vi "Func - Get list of string arguments.vi"(5 "InstanceRef":T1, 6 "error in":bool, 7 "max arg num":i32=100, 8 "min arg num":i32=1, 9 "arg list":T2[](array[typedef])) -> (0 "error out":bool, 3 "val list":string[](array[string]))   [LabVIEW 2021]
doc: "This VI returns the values of function arguments which must all have the <b>String</b> data type. It verifies the number of actual arguments and their data types. Refer to the VI help for more details.\n\n<b>arg list</b> specifies the list of function arguments passed to a FuncVI. Wire it to the same terminal on the FuncVI block diagram.\n\n<b>min arg num</b> and <b>max arg num</b> specify the minimum and the maximum number of arguments allowed.\n\n::: CalcExpress Toolkit :::\nCopyright (c) 2000-2026 Konstantin Shifershteyn. All rights reserved."
uses:
  cetypes.llb/CalcExpress Function Argument Info.ctl
  cetypes.llb/CalcExpress Instance RefNum.ctl
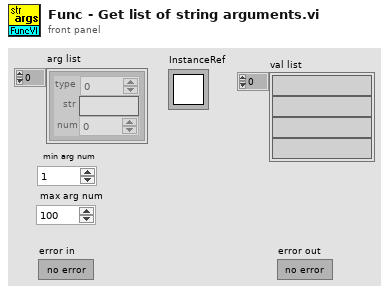
[diagram p1: front panel]
types:
  T1 = typedef "CalcExpress Instance RefNum.ctl" = refnum<k1>
  T2 = typedef "CalcExpress Function Argument Info.ctl" = cluster{"type":u32, "str":string, "num":dbl}
  T3 = enum32{"String", "DBL Number", "identifier", "1D Array of DBL", "2D Array of DBL", "CDB Number", "1D Array of CDB", "2D Array of CDB", "1D Array of String", "2D Array of String", "Unknown data type"}
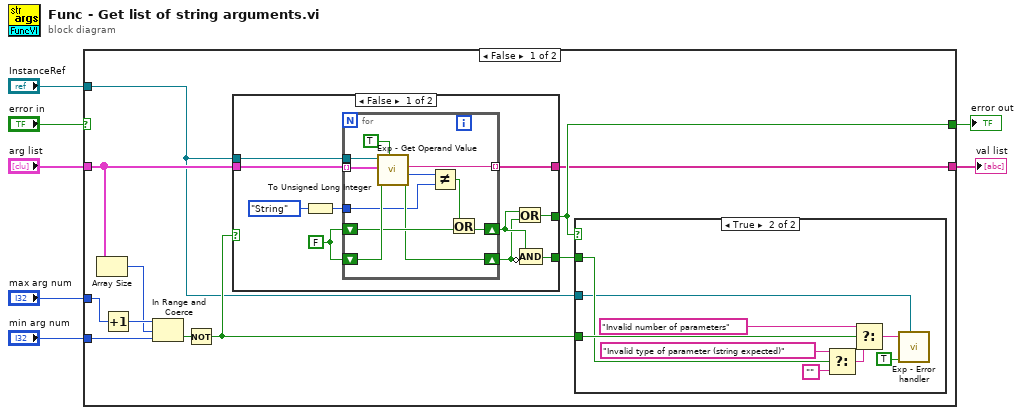
[diagram p0: block diagram]
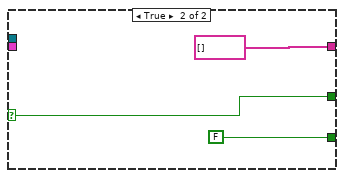
[diagram p2: hidden frame]
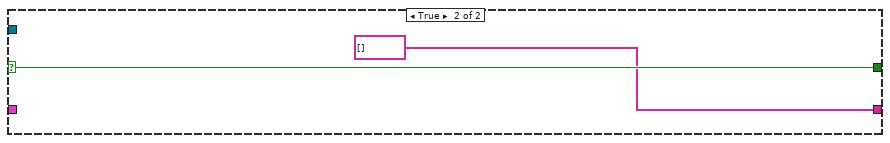
[diagram p4: hidden frame]
diagram:
  n1 = case shown="False" "error in" {
    selector: "error in" -> [_ w53]
    tunnel: [w13 w53] -> w7
    tunnel: [w12 string[] []] -> w6
    tunnel: "InstanceRef" -> [w8 _]
    tunnel: "arg list" -> [w11 _]
    tunnel: "min arg num" -> [w10 _]
    tunnel: "max arg num" -> [w9 _]
    frame False {
      n2 = Array Size(array=w11) -> (size(s)=w15:i32)
      n3 = Increment(x=w9) -> (x+1=w16:i32)
      n4 = In Range and Coerce(upper limit=w16, x=w15, lower limit=w10) -> (In Range?=w14:bool)  [unwired: 1 out]
      n5 = Not(x=w14) -> (.not. x?=w18:bool)
      n6 = case shown="False" w18 {
        selector: w18 -> [_ w42]
        tunnel: w11 -> [w25 _]
        tunnel: [w24 w42] -> w13
        tunnel: [w23 FALSE] -> w17
        tunnel: w8 -> [w22 _]
        tunnel: [w21 string[] []] -> w12
        frame False {
          w28 = FALSE
          n7 = To Unsigned Long Integer(number=T3."String" ("data type")) -> (unsigned 32bit integer=w19:u32)
          n8 = for {
            tunnel: w25 -> [w33] mode=indexing
            shift-right: [w35] -> w26
            shift-left: w28 -> [w38]
            shift-right: [w36] -> w27
            shift-left: w28 -> [w37]
            tunnel: [w34] -> w21 mode=indexing
            tunnel: w22 -> [w32]
            tunnel: w19 -> [w29]
            n9 = call "Exp - Get Operand Value.vi"("ena string? (F)"=TRUE ("may be string ? (F)"), "error in"=w38, "op info"=w33, "InstanceRef"=w32) -> ("error out"=w35:bool, "type"=w31:u32, "str"=w34:string)  [unwired: 2 in, 1 out]
            n10 = Not Equal?(x=w31, y=w29) -> (x != y?=w30:bool)
            n11 = Or(x=w30, y=w37) -> (x .or. y?=w36:bool)
          }
          n12 = Or(x=w27, y=w26) -> (x .or. y?=w24:bool)
          n13 = Compound Arithmetic op=AND(w27, invert w26) -> (w23:bool)
        }
        frame True {
        }
      }
      n14 = case shown="True" w13 {
        tunnel: w18 -> [_ w51]
        tunnel: w17 -> [_ w49]
        tunnel: w8 -> [_ w43]
        frame False {
        }
        frame True {
          n15 = Select(t="Invalid type of parameter (string expected)" ("ErrStr"), s=w49, f="" ("Empty String Constant")) -> (s? t:f=w46:string)
          n16 = Select(t="Invalid number of parameters" ("ErrStr"), s=w51, f=w46) -> (s? t:f=w44:string)
          n17 = call "Exp - Error handler.vi"("InstanceRef"=w43, "error in"=TRUE, "error message in"=w44) -> ()  [unwired: 6 in, 3 out]
        }
      }
    }
    frame True {
    }
  }
  "error out" <- w7
  "val list" <- w6
